vi "Close.vi"(8 "error in (no error)":errorcluster, 11 "Data in":refnum<class "CTI_Bus.lvclass">) -> (0 "error out":errorcluster, 3 "Data out":refnum<class "CTI_Bus.lvclass">)   [LabVIEW 2021, in "CTI_Bus.lvclass"]
doc: "Abstract Data Classes 2.1.1.13\nTim Streeter - TSA\nCopyright (c) 2025, TSA"
uses:
  CTI_Bus.lvclass
  CTI_Bus.lvclass/CTI_Bus.ctl
  <vilib>/CTI/CTI Drivers/CTI/Session/Session.lvclass
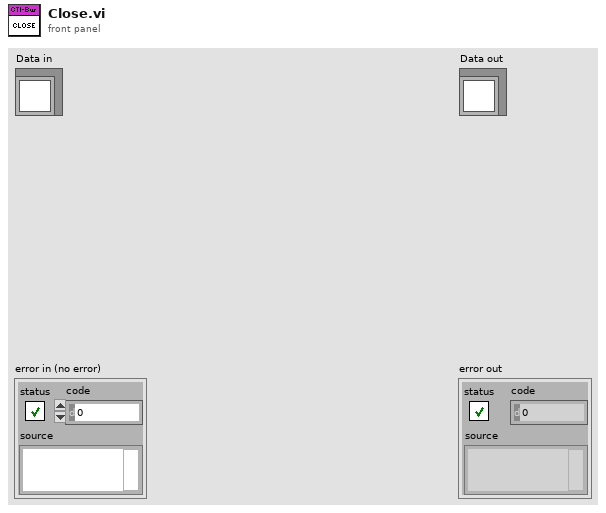
[diagram p1: front panel]
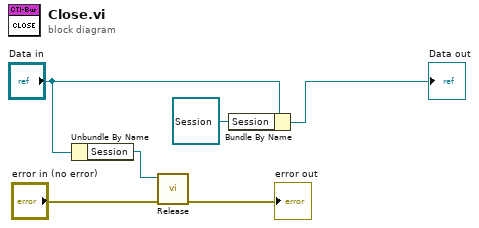
[diagram p0: block diagram]
diagram:
  n1 = Unbundle By Name("Data in") -> ("Session"=w5:refnum<class "Session.lvclass">)
  n2 = call-dynamic "Release.vi"("error in (no error)"="error in (no error)", "Session in"=w5) -> ("error out"=→"error out":errorcluster)  [unwired: 9 in]
  n3 = Bundle By Name(cluster="Data in", "Session"=refnum<class "Session.lvclass"> refnum) -> (→"Data out":refnum<class "CTI_Bus.lvclass">)
